vi "Get ILP.vi"(6 "Color":T1, 7 "OLED-PD dist":dbl, 8 "error in (no error)":errorcluster, 9 "DAQ V":dbl, 10 "OLED A":dbl, 11 "Acquistion Data":T2) -> (0 "error out":errorcluster, 3 "Acquistion Data":T2)   [LabVIEW 2020]
uses:
  controls/Acquisition data --typedef.ctl
  controls/Color --typedef.ctl
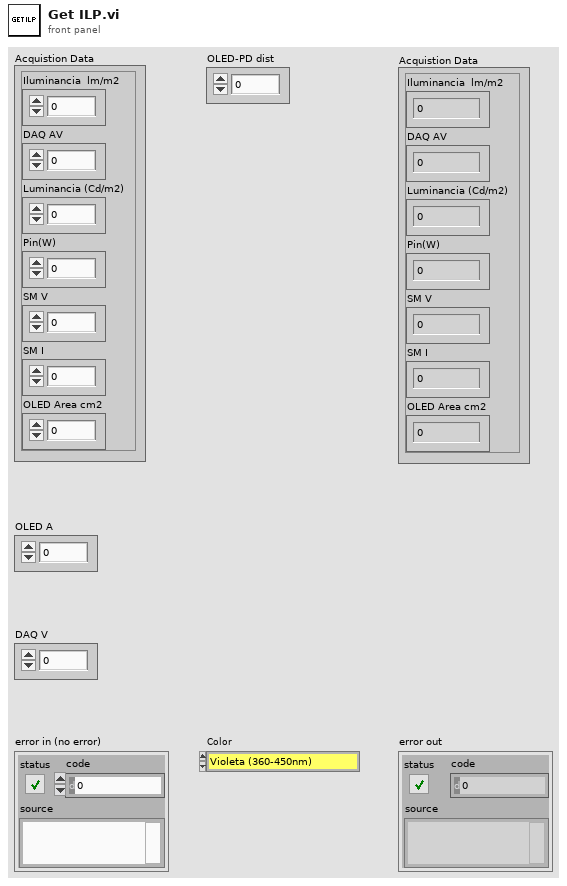
[diagram p1: front panel]
types:
  T1 = typedef "Color --typedef.ctl" = enum16{"Violeta (360-450nm)", "Azul (450-500nm)", "Verde(500-570nm)", "Amarillo (570-590nm)", "Naranja (600-610nm)", "Rojo (610-670nm)", "Blanco"}
  T2 = typedef "Acquisition data --typedef.ctl" = cluster{"Iluminancia  lm/m2":dbl, "DAQ AV":dbl, "Luminancia (Cd/m2)":dbl, "Pin(W)":dbl, "SM V":dbl, "SM I":dbl, "OLED Area cm2":dbl}
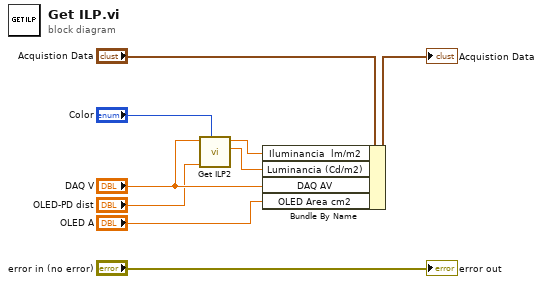
[diagram p0: block diagram]
diagram:
  n1 = call "Get ILP2.vi"("Color"="Color", "S (Distancia OLED-fotodiodo) cm"="OLED-PD dist", "x (volts)"="DAQ V") -> ("Luminancia (Cd/m2)"=w3:dbl, "Iluminancia  lm/m2"=w4:dbl)  [unwired: 7 in]
  n2 = Bundle By Name(cluster="Acquistion Data", "Iluminancia  lm/m2"=w4, "Luminancia (Cd/m2)"=w3, "DAQ AV"="DAQ V", "OLED Area cm2"="OLED A") -> (→"Acquistion Data":T2)
  "error out" <- "error in (no error)"
